vi "call async imaq save.vi"(7 "Status":T1, 8 "error in (no error)":errorcluster, 9 "Boolean":bool, 10 "Refnum in":T2, 11 "FakeCamera in":refnum<class "Point Grey Camera.lvclass">) -> (0 "error out":errorcluster, 3 "FakeCamera out":refnum<class "Point Grey Camera.lvclass">)   [LabVIEW 2020, in "Point Grey Camera.lvclass"]
uses:
  Point Grey Camera.lvclass
  IMAQ Image.ctl
  1st or last shot of scan.ctl
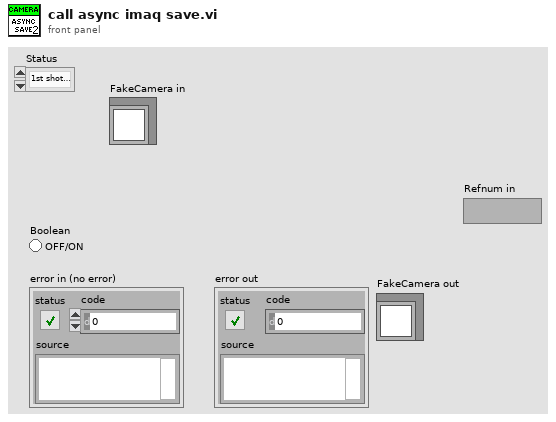
[diagram p1: front panel]
types:
  T1 = typedef "1st or last shot of scan.ctl" = enum16{"1st shot of scan", "1st shot after scan end", "other"}
  T2 = typedef "IMAQ Image.ctl" = refnum<image>
  T3 = typedef "Image Type" = u32
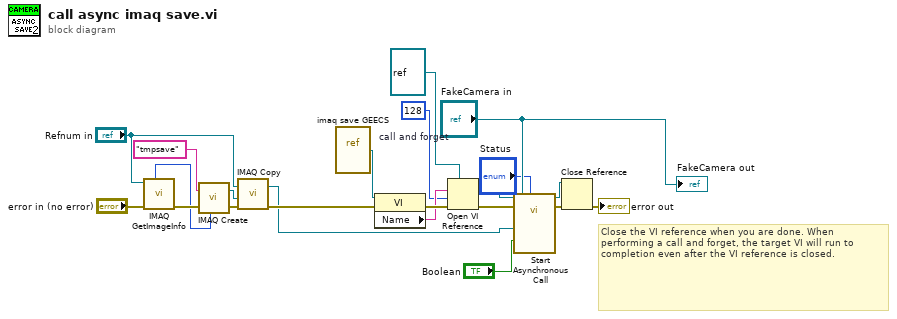
[diagram p0: block diagram]
diagram:
  w8 = 128  # call and forget
  # "Close the VI reference when you are done. When performing a call and forget, the target VI will run to completion even after the VI reference is closed."
  n1 = call "IMAQ GetImageInfo"("error in (no error)"="error in (no error)", "Image"="Refnum in") -> ("error out"=w20:errorcluster, "Image Type"=w5:T3)  [unwired: 2 in, 6 out]
  n2 = call "IMAQ Create"("Image Name"="tmpsave", "Image Type"=w5, "error in (no error)"=w20) -> ("New Image"=w6:T2, "error out"=w21:errorcluster)  [unwired: 2 in]
  n3 = call "IMAQ Copy"("error in (no error)"=w21, "Image Dst"=w6, "Image Src"="Refnum in") -> ("error out"=w22:errorcluster, "Image Dst Out"=w3:T2)  [unwired: 3 in]
  n4 = vi-ref "imaq save GEECS.vi"() -> (w14:refnum<vi>)
  n5 = property class="VI"(reference=w14, error in=w22) -> (error out=w16:errorcluster, "Name"=w15:string)  [unwired: 1 out]
  n6 = Open VI Reference(type specifier VI Refnum (for type only)=refnum<vi> refnum, vi path=w15, options=w8, error in (no error)=w16) -> (vi reference=w10:refnum<vi>, error out=w11:errorcluster)  [unwired: 2 in]
  n7 = call-by-ref "Start Asynchronous Call"(reference=w10, error in=w11, "Status"="Status", "file already written"="Boolean", "Refnum in"=w3, "FakeCamera in"="FakeCamera in") -> (reference out=w13:refnum<vi>, error out=w12:errorcluster)  [unwired: 6 in, 2 out]
  n8 = Close Reference(reference=w13, error in (no error)=w12) -> (error out=→"error out":errorcluster)
  "FakeCamera out" <- "FakeCamera in"
